vi "Initialize.vi"(8 "error in":errorcluster, 10 "shared resources":refnum<class "Shared Resources.lvclass">, 11 "Ballard ARINC-429 Tx Execution Unit in":refnum<class "Tx Scheduled Labels Execution Unit.lvclass">) -> (0 "error out":errorcluster, 3 "Ballard ARINC-429 Tx Execution Unit out":refnum<class "Tx Scheduled Labels Execution Unit.lvclass">)   [LabVIEW 2020, in "Ballard ARINC 429 Engine.lvlib" / "Implementation.lvlib" / "Tx Scheduled Labels Execution Unit.lvclass"]
uses:
  Tx Scheduled Labels Execution Unit.lvclass
  C:/git/ni/niveristand-ballard-arinc429-custom-device/Source/Custom Device Support/Engine/Implementation/Execution Unit/Execution Unit.lvclass
  Interfaces/Shared Resources/Shared Resources.lvclass
  Shared Resources/Shared Resources.lvclass
  Shared Resources/Shared Resources.lvclass/Shared Resources.ctl
  Execution Unit/Execution Unit.lvclass/Execution Unit.ctl
  Tx Scheduled Labels Execution Unit.lvclass/Tx Scheduled Labels Execution Unit.ctl
  <instrlib>/BTI429Lib/BTI429LV.lvlib
  Custom Device/Custom Device.lvlib
  Execution Unit/Execution Unit.lvclass
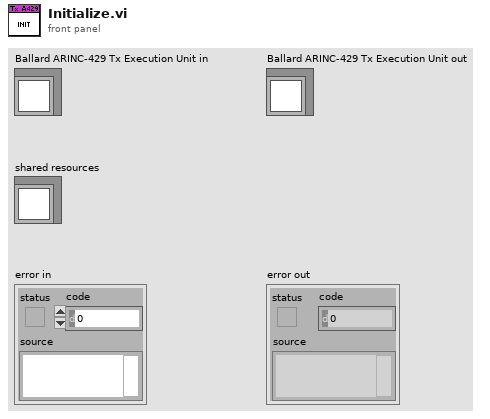
[diagram p1: front panel]
types:
  T1 = typedef "Ballard ARINC 429 Engine.lvlib/Custom Device.lvlib/Hardware Handles.ctl" = cluster{"core handle":u64, "core reader handle":u64, "channel handles":u64[]}
  T2 = typedef "RT Hardware Channel Settings.ctl" = cluster{"channel #":u16, "channel handle":u64, "labels settings for RT":T3[]}
  T3 = typedef "RT Label Settings.ctl" = cluster{"Name":string, "xmlName":string, "label":T4, "transfer period":u32, "SDI_Enabled":bool, "SDI":u8, "parameter driver data":T5, "transfer type":T9, "has timestamp?":bool, "Label Disable/Trigger Channel Reference":T8, "Message Handle":u64, "Initialized?":bool, "Word Initial Raw Value":u32, "Label Timestamp Channel Data Reference":T10, "disabled":bool}
  T4 = typedef "Label.ctl" = u8
  T5 = typedef "RT Parameters.ctl" = cluster{"parameter definitions":T6[], "Tx parameter refs":T8[]}
  T6 = typedef "Parameter Definition.ctl" = cluster{"start index":i32, "size":i32, "encoding":T7, "signed":bool, "scale multiplier":dbl, "scale offset":dbl}
  T7 = typedef "Encoding and Decoding.lvlib/Encoding.ctl" = enum16{"BNR", "BCD", "Discrete"}
  T8 = typedef "Custom Device API.lvlib/Custom Device Item Ref.ctl" = u64
  T9 = typedef "Transfer Type.ctl" = enum16{"Scheduled", "Acyclic", "Block", "Strobe"}
  T10 = typedef "Custom Device API.lvlib/Data Reference.ctl" = i32
  T11 = typedef "Map of Values Indexes to Channel and Label Indexes.ctl" = map{i32, cluster{"channel index":i32, "label index":i32, "group values start index":i32, "values in group":i32}}
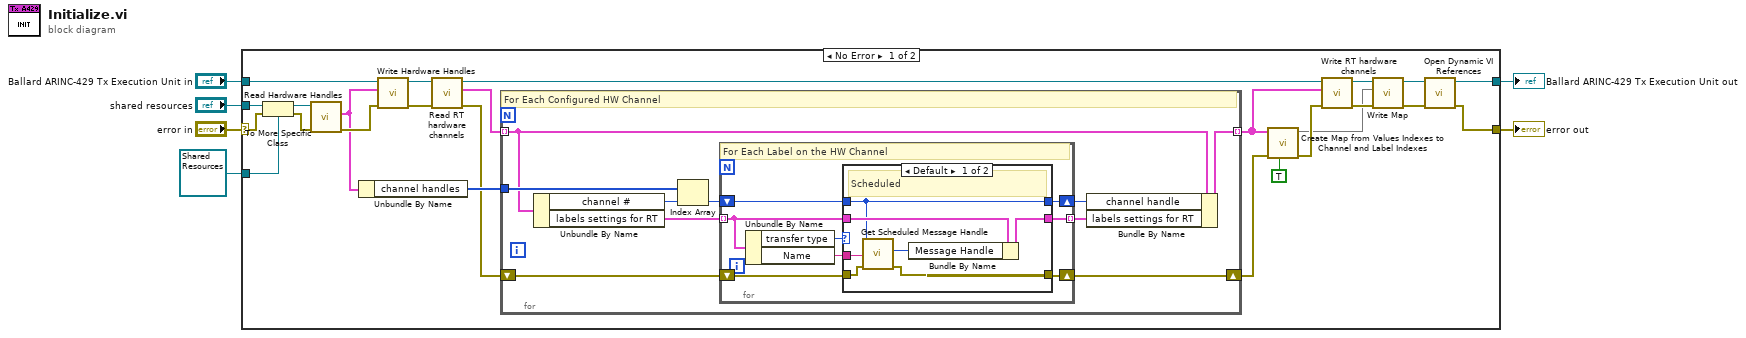
[diagram p0: block diagram]
diagram:
  n1 = case shown="No Error" "error in" {
    selector: "error in" -> [w16 w60]
    tunnel: "Ballard ARINC-429 Tx Execution Unit in" -> [w20 w61]
    tunnel: [w8 w61] -> w5
    tunnel: [w7 w60] -> w3
    tunnel: "shared resources" -> [w14 _]
    tunnel: refnum<class "Shared Resources.lvclass"> refnum ("Ballard ARINC-429 shared resources in") -> [w13 _]
    frame No Error {
      n2 = To More Specific Class(target class=w13, reference=w14, error in=w16) -> (specific class reference=w12:refnum<class "Shared Resources.lvclass">, error out=w15:errorcluster)
      n3 = call "Read Hardware Handles.vi"("error in"=w15, "Ballard ARINC-429 shared resources in"=w12) -> ("error out"=w21:errorcluster, "hardware handles"=w18:T1)  [unwired: 7 in, 1 out]
      n4 = Unbundle By Name(w18) -> ("channel handles"=w31:u64[])
      n5 = call "Write Hardware Handles.vi"("error in"=w21, "hardware handles"=w18, "Ballard ARINC-429 Execution Unit in"=w20) -> ("error out"=w17:errorcluster, "Ballard ARINC-429 Execution Unit out"=w19:refnum<class "Tx Scheduled Labels Execution Unit.lvclass">)  [unwired: 7 in]
      n6 = call "Read RT hardware channels.vi"("error in"=w17, "Ballard ARINC-429 Tx Execution Unit in"=w19) -> ("error out"=w28:errorcluster, "RT hardware channels"=w30:T2[], "Ballard ARINC-429 Tx Execution Unit out"=w29:refnum<class "Tx Scheduled Labels Execution Unit.lvclass">)  [unwired: 7 in]
      n7 = for {
        shift-right: [w32] -> w26
        shift-left: w28 -> [w37]
        tunnel: w30 -> [w36] mode=indexing
        tunnel: w31 -> [w40]
        tunnel: [w33] -> w27 mode=indexing
        # "For Each Configured HW Channel"
        n8 = Unbundle By Name(w36) -> ("channel #"=w41:u16, "labels settings for RT"=w38:T3[])
        n9 = Index Array(array=w40, index=w41) -> (element=w39:u64)
        n10 = for {
          tunnel: w38 -> [w44] mode=indexing
          shift-right: [w45] -> w32
          shift-left: w37 -> [w46]
          tunnel: [w43] -> w35 mode=indexing
          shift-right: [w42] -> w34
          shift-left: w39 -> [w48]
          # "For Each Label on the HW Channel"
          n11 = Unbundle By Name(w44) -> ("transfer type"=w49:T9, "Name"=w47:string)
          n12 = case shown="Default" w49 {
            tunnel: w48 -> [w50 w57]
            tunnel: w47 -> [w56 _]
            tunnel: w46 -> [w55 w59]
            tunnel: [w54 w59] -> w45
            tunnel: w44 -> [w52 w58]
            tunnel: [w51 w58] -> w43
            tunnel: [w50 w57] -> w42
            frame Default {
              # "Scheduled"
              n13 = call <instrlib>:"Get Scheduled Message Handle.vi"("error in (no error)"=w55, "message name"=w56, "channel handle in"=w50) -> ("error out"=w54:errorcluster, "message handle out"=w53:u64)  [unwired: 6 in, 1 out]
              n14 = Bundle By Name(cluster=w52, "Message Handle"=w53) -> (w51:T3)
            }
            frame "Acyclic" {
            }
          }
        }
        n15 = Bundle By Name(cluster=w36, "channel handle"=w34, "labels settings for RT"=w35) -> (w33:T2)
      }
      n16 = call "Create Map from Values Indexes to Channel and Label Indexes.vi"("disable channel included in group"=TRUE, "error in"=w26, "RT hardware channels"=w27) -> ("error out"=w25:errorcluster, "map from values index to RT info indexes"=w22:T11)  [unwired: 7 in]
      n17 = call "Write RT hardware channels.vi"("error in"=w25, "RT hardware channels"=w27, "Ballard ARINC-429 Tx Execution Unit in"=w29) -> ("error out"=w24:errorcluster, "Ballard ARINC-429 Tx Execution Unit out"=w23:refnum<class "Tx Scheduled Labels Execution Unit.lvclass">)  [unwired: 7 in]
      n18 = call "Write Map.vi"("error in"=w24, "map from values indexes to RT info indexes"=w22, "Ballard ARINC-429 Tx Execution Unit in"=w23) -> ("error out"=w10:errorcluster, "Ballard ARINC-429 Tx Execution Unit out"=w9:refnum<class "Tx Scheduled Labels Execution Unit.lvclass">)  [unwired: 7 in]
      n19 = call-dynamic "Open Dynamic VI References.vi"("error in (no error)"=w10, "Tx Scheduled Labels Execution Unit in"=w9) -> ("error out"=w7:errorcluster, "Tx Scheduled Labels Execution Unit out"=w8:refnum<class "Tx Scheduled Labels Execution Unit.lvclass">)  [unwired: 8 in]
    }
    frame Error {
    }
  }
  "error out" <- w3
  "Ballard ARINC-429 Tx Execution Unit out" <- w5
